vi "D4xxx Set Output mode.vi"(7 "error in":errorcluster, 9 "Output mode (0:Standby)":u16(ring) items=["Standby", "Operate"], 10 "4808":refnum<visa-resource-name>) -> (0 "error out":errorcluster, 3 "Session Out":refnum<visa-resource-name>)   [LabVIEW 2011]
doc: "Set output on or off of Datron 4xxx series calibrators."
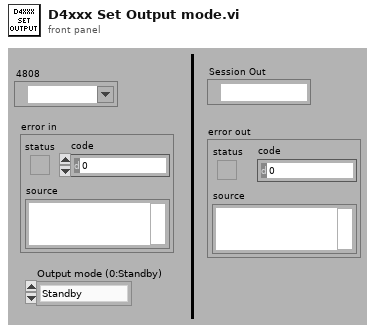
[diagram p1: front panel]
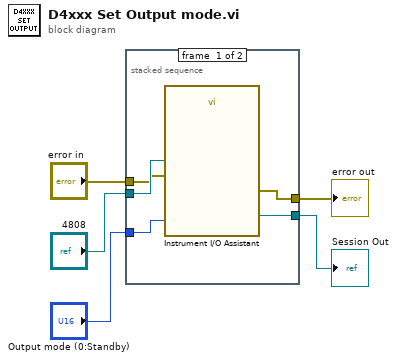
[diagram p0: block diagram]
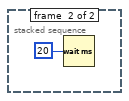
[diagram p2: hidden frame]
diagram:
  n1 = stacked-sequence {
    tunnel: "4808" -> [w10 _]
    tunnel: [w9 _] -> w3
    tunnel: [w8 _] -> w4
    tunnel: "error in" -> [w7 _]
    tunnel: "Output mode (0:Standby)" -> [w6 _]
    frame #0 {
      n2 = call "Instrument I/O Assistant"("Session In"=w10, "OPR"=w6, "error in"=w7) -> ("Session Out"=w8:refnum<visa-resource-name>, "error out"=w9:errorcluster)  [unwired: 23 in]
    }
    frame #1 {
      n3 = Wait (ms)(milliseconds to wait=u32 20 ("millisecond multiple")) -> ()  [unwired: 1 out]
    }
  }
  "Session Out" <- w4
  "error out" <- w3
